vi "Import Export - Export to XML File.vi"(8 "error in":errorcluster, 10 "Configuration File Path":path, 11 "Item Ref in":T1 format="%.0x") -> (0 "error out":errorcluster, 3 "Item Ref out":T1 format="%.0x", 4 "xml string":string)   [LabVIEW 2017, in "PXImc System Explorer.lvlib"]
uses:
  PXImc System Explorer.lvlib
  <vilib>/NI Veristand/Custom Device API/Custom Device Item Ref.ctl
  <vilib>/NI/NI VeriStand Custom Device Import and Export Tool/ImportExport.lvlib
  <vilib>/NI VeriStand/Custom Device API/Custom Device API.lvlib
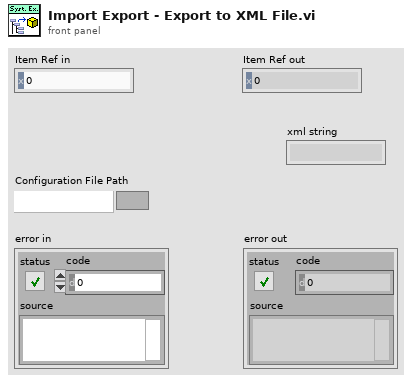
[diagram p1: front panel]
types:
  T1 = typedef "Custom Device API.lvlib/Custom Device Item Ref.ctl" = u64
  T2 = typedef "Advanced System Definition.lvlib/SysDef.Export.ctl" = cluster{"Version":string, "Tree":T3[]}
  T3 = typedef "Advanced System Definition.lvlib/TreeItem.ctl" = cluster{"Item Info":T4, "Parent Path":string[], "Properties":T9[]}
  T4 = typedef "Advanced System Definition.lvlib/TreeItem.Info.ctl" = cluster{"Name":string, "Description":string, "GUID":string, "Is Channel":bool, "Channel":T5, "Is Waveform":bool, "Waveform":T7}
  T5 = typedef "Custom Device API.lvlib/Custom Device Channel.ctl" = cluster{"Type":T6, "Units":string, "Default Value":dbl, "Faultable":bool, "Scalable":bool}
  T6 = typedef "Custom Device API.lvlib/Custom Device Channel Type.ctl" = enum16{"Input", "Output"}
  T7 = typedef "Custom Device API.lvlib/Custom Device Waveform.ctl" = cluster{"Data Type":T8, "Units":string}
  T8 = typedef "Custom Device API.lvlib/Custom Device Waveform DataType.ctl" = enum16{"Double", "Complex Double"}
  T9 = typedef "Advanced System Definition.lvlib/TreeItem.Property.ctl" = cluster{"Name":string, "Type":i32, "Value":variant}
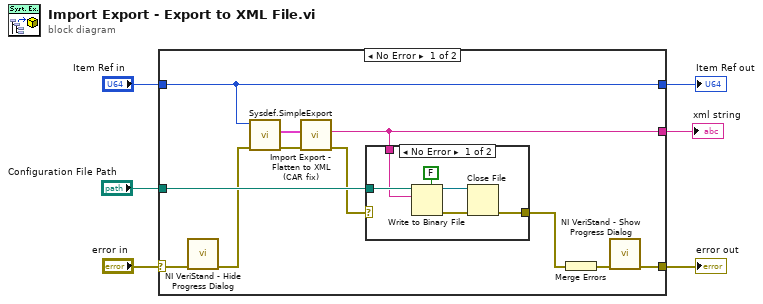
[diagram p0: block diagram]
diagram:
  n1 = case shown="No Error" "error in" {
    selector: "error in" -> [w10 w25]
    tunnel: [w7 w25] -> w5
    tunnel: [w17 w26] -> w4
    tunnel: "Item Ref in" -> [w17 w26]
    tunnel: "Configuration File Path" -> [w16 _]
    tunnel: [w14 _] -> w1
    frame No Error {
      n2 = call <vilib>:"NI VeriStand - Hide Progress Dialog.vi"("error in (no error)"=w10) -> ("error out"=w9:errorcluster)  [unwired: 10 in]
      n3 = call <vilib>:"Sysdef.SimpleExport.vi"("error in (no error)"=w9, "ID"=w17) -> ("error out"=w13:errorcluster, "Export"=w11:T2)  [unwired: 7 in, 1 out]
      n4 = call "Import Export - Flatten to XML (CAR fix).vi"("Error In"=w13, "Export"=w11) -> ("Error Out"=w12:errorcluster, "XML String Out"=w14:string)  [unwired: 8 in]
      n5 = case shown="No Error" w12 {
        selector: w12 -> [_ w24]
        tunnel: w16 -> [w20 _]
        tunnel: w14 -> [w18 _]
        tunnel: [w22 w24] -> w15
        frame No Error {
          n6 = Write to Binary File(file (use dialog)=w20, data=w18, 5:FALSE ("prepend array or string size? (T)")) -> (refnum out=w23:refnum<file>, error out=w21:errorcluster)  [unwired: 1 in, 3 out]
          n7 = Close File(refnum=w23, error in=w21) -> (error out=w22:errorcluster)  [unwired: 1 out]
        }
        frame Error {
        }
      }
      n8 = Merge Errors(w15) -> (w8:errorcluster)
      n9 = call <vilib>:"NI VeriStand - Show Progress Dialog.vi"("error in (no error)"=w8) -> ("error out"=w7:errorcluster)  [unwired: 10 in]
    }
    frame Error {
    }
  }
  "error out" <- w5
  "Item Ref out" <- w4
  "xml string" <- w1
